vi "US Check rightside.vi"   [LabVIEW 2017]
uses:
  <instrlib>/Parallax PING)))/FPGA/NI_Robotics_Parallax PING))) (FPGA).lvlib
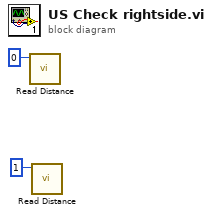
[diagram p0: block diagram]
diagram:
  n1 = call <instrlib>:"Read Distance.vi"("sensor ID"=i16 0) -> ()  [unwired: 9 in, 2 out]
  n2 = call <instrlib>:"Read Distance.vi"("sensor ID"=i16 1) -> ()  [unwired: 9 in, 2 out]
